vi "Scripting_AlignToConenctorPane.vi"(8 "error in":errorcluster, 11 "ViRef In":refnum<vi>) -> (0 "error out":errorcluster, 3 "VIRefOut":refnum<vi>)   [LabVIEW 2020, in "Scripting.lvclass"]
uses:
  <resource>/Framework/Providers/Open_GDS/ClassProviders/Common/ScriptingFunctions/Scripting.lvclass
  <resource>/Framework/Providers/Open_GDS/ClassProviders/Common/ScriptingFunctions/Scripting.lvclass/Scripting.ctl
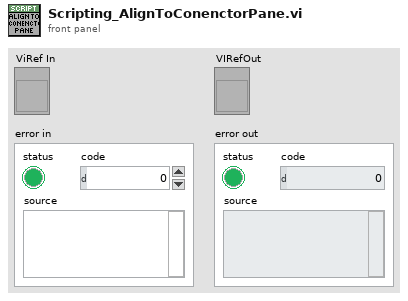
[diagram p1: front panel]
types:
  T1 = enum32{"Top Edges", "Vertical Centers", "Bottom Edges", "Left Edges", "Horizontal Centers", "Right Edges"}
  T2 = typedef "LVRectTypeDef.ctl" = cluster{"Left":i16, "Top":i16, "Right":i16, "Bottom":i16}
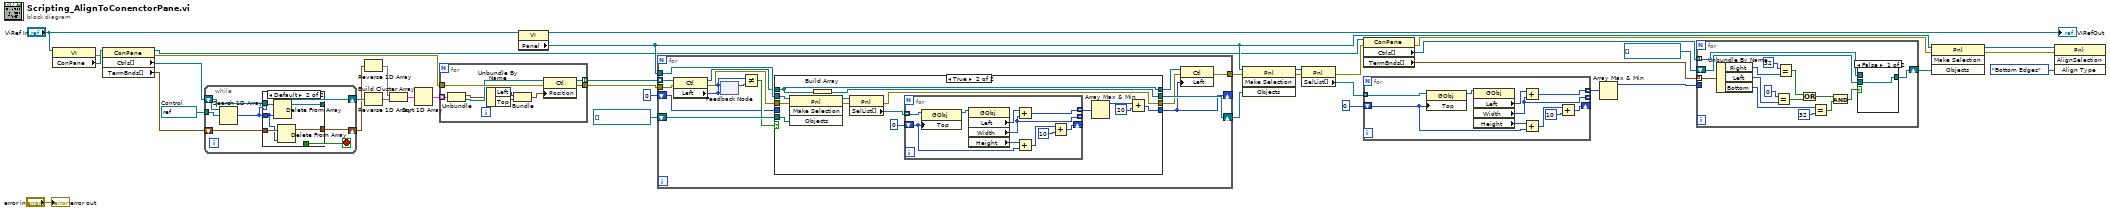
[diagram p0: block diagram]
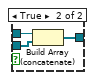
[diagram p2: hidden frame]
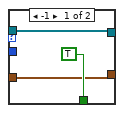
[diagram p3: hidden frame]
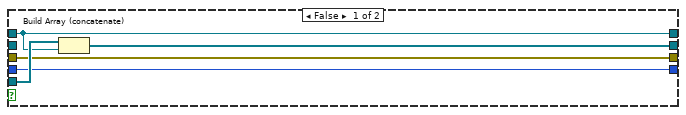
[diagram p4: hidden frame]
diagram:
  w17 = refnum<vi> refnum  # Control
  n1 = property class="VI"(reference="ViRef In") -> (error out=w28:errorcluster, "ConPane"=w33:refnum<vi>)  [unwired: 1 in, 1 out]
  n2 = property class="ConPane"(reference=w33, error in=w28) -> (reference out=w29:refnum<vi>, error out=w24:errorcluster, "Ctrls[]"=w36:refnum<vi>[], "TermBnds[]"=w35:T2[])
  n3 = while {
    tunnel: w17 -> [w39]
    shift-right: [w44] -> w27
    shift-left: w36 -> [w45]
    shift-right: [w40] -> w26
    shift-left: w35 -> [w41]
    stop <- w42 stop-if-true
    n4 = Search 1D Array(1D array=w45, element=w39) -> (index of element=w43:i32)  [unwired: 1 in]
    n5 = case shown="Default" w43 {
      tunnel: w43 -> [_ w49]
      tunnel: w45 -> [w48 w53]
      tunnel: [w48 w52] -> w44
      tunnel: [TRUE _] -> w42
      tunnel: w41 -> [w46 w51]
      tunnel: [w46 w50] -> w40
      frame -1 {
      }
      frame Default {
        n6 = Delete From Array(array=w53, index=w49) -> (array with subset deleted=w52:refnum<vi>[])  [unwired: 1 in, 1 out]
        n7 = Delete From Array(array=w51, index=w49) -> (array with subset deleted=w50:T2[])  [unwired: 1 in, 1 out]
      }
    }
  }
  n8 = Reverse 1D Array(array=w26) -> (reversed array=w21:T2[])
  n9 = Reverse 1D Array(array=w27) -> (reversed array=w20:refnum<vi>[])
  n10 = Build Cluster Array(w21, w20) -> (w19:cluster{"Rectangle":T2, refnum<vi>}[])
  n11 = Sort 1D Array(array=w19) -> (sorted array=w18:cluster{"Rectangle":T2, refnum<vi>}[])
  n12 = for {
    tunnel: [w59] -> w37 mode=indexing
    tunnel: [w58] -> w30
    tunnel: w24 -> [w57]
    tunnel: w18 -> [w56] mode=indexing
    n13 = Unbundle(w56) -> ("Rectangle"=w54:T2, w55:refnum<vi>)
    n14 = Unbundle By Name(w54) -> ("Left"=w62:i16, "Top"=w61:i16)
    n15 = Bundle("Left"=w62, "Top"=w61) -> (w60:cluster{"Left":i16, "Top":i16})  [unwired: 1 in]
    n16 = property class="Ctl"(reference=w55, error in=w57, "Position"=w60) -> (reference out=w59:refnum<vi>, error out=w58:errorcluster)
  }
  n17 = property class="VI"(reference="ViRef In") -> (reference out=→"VIRefOut":refnum<vi>, "Panel"=w32:refnum<vi>)  [unwired: 1 in, 1 out]
  n18 = for {
    shift-right: [w76] -> w22
    shift-left: refnum<vi>[] [] -> [w75]
    shift-right: [w69] -> _
    shift-left: u32 0 ("Numeric") -> [w70]
    tunnel: w32 -> [w74]
    tunnel: w37 -> [w73] mode=indexing
    tunnel: [w67] -> w31
    tunnel: w30 -> [w65]
    n19 = property class="Ctl"(reference=w73, error in=w65) -> (reference out=w64:refnum<vi>, error out=w66:errorcluster, "Left"=w71:i32)
    n20 = feedback-in #1(w71) -> ()
    n21 = feedback #1(w71) -> (w77:i32)
    n22 = Not Equal?(x=w71, y=w77) -> (x != y?=w72:bool)
    n23 = case shown="True" w72 {
      tunnel: [w82 w96] -> w76
      tunnel: w75 -> [w81 w94]
      tunnel: [w80 w89] -> w69
      tunnel: w74 -> [_ w95]
      tunnel: w70 -> [w80 _]
      tunnel: [w79 w93] -> w68
      tunnel: w66 -> [w79 w92]
      tunnel: w64 -> [w78 w91]
      tunnel: [w78 w91] -> w63
      frame False {
        n24 = Build Array (concatenate)(w81, w78) -> (w82:refnum<vi>[])
      }
      frame True {
        n25 = invoke class="Pnl" method="Make Selection"(reference=w95, error in=w92, "Objects"=w94) -> (reference out=w87:refnum<vi>, error out=w86:errorcluster)  [unwired: 1 in, 2 out]
        n26 = Build Array(w91) -> (w96:refnum<vi>[])
        n27 = property class="Pnl"(reference=w87, error in=w86) -> (error out=w93:errorcluster, "SelList[]"=w84:refnum<vi>[])  [unwired: 1 out]
        n28 = for {
          tunnel: w84 -> [w99] mode=indexing
          tunnel: [w106] -> w83 mode=indexing
          tunnel: [w105] -> _ mode=indexing
          shift-right: [w100] -> _
          shift-left: u32 0 -> [w97]
          n29 = property class="GObj"(reference=w99, "Top"=w97) -> (reference out=w98:refnum<vi>)  [unwired: 1 in, 1 out]
          n30 = property class="GObj"(reference=w98) -> ("Left"=w104:i32, "Width"=w105:u32, "Height"=w103:u32)  [unwired: 1 in, 2 out]
          n31 = Add(x=w104, y=w105) -> (x+y=w106:u32)
          n32 = Add(x=w103, y=w97) -> (x+y=w102:u32)
          n33 = Add(x=w102, y=u32 10) -> (x+y=w100:u32)
        }
        n34 = Array Max & Min(array=w83) -> (max value=w90:u32)  [unwired: 3 out]
        n35 = Add(x=w90, y=u32 20) -> (x+y=w89:u32)
      }
    }
    n36 = property class="Ctl"(reference=w63, error in=w68, "Left"=w69) -> (error out=w67:errorcluster)  [unwired: 1 out]
  }
  n37 = invoke class="Pnl" method="Make Selection"(reference=w32, error in=w31, "Objects"=w22) -> (reference out=w16:refnum<vi>, error out=w15:errorcluster)  [unwired: 1 in, 2 out]
  n38 = property class="Pnl"(reference=w16, error in=w15) -> (error out=w3:errorcluster, "SelList[]"=w13:refnum<vi>[])  [unwired: 1 out]
  n39 = property class="ConPane"(reference=w29, error in=w3) -> (error out=w4:errorcluster, "Ctrls[]"=w11:refnum<vi>[], "TermBnds[]"=w10:T2[])  [unwired: 1 out]
  n40 = for {
    tunnel: w13 -> [w109] mode=indexing
    tunnel: [w116] -> w12 mode=indexing
    tunnel: [w115] -> _ mode=indexing
    shift-right: [w110] -> _
    shift-left: u32 0 -> [w107]
    n41 = property class="GObj"(reference=w109, "Top"=w107) -> (reference out=w108:refnum<vi>)  [unwired: 1 in, 1 out]
    n42 = property class="GObj"(reference=w108) -> ("Left"=w114:i32, "Width"=w115:u32, "Height"=w113:u32)  [unwired: 1 in, 2 out]
    n43 = Add(x=w114, y=w115) -> (x+y=w116:u32)
    n44 = Add(x=w113, y=w107) -> (x+y=w112:u32)
    n45 = Add(x=w112, y=u32 10) -> (x+y=w110:u32)
  }
  n46 = Array Max & Min(array=w12) -> (max value=w2:u32)  [unwired: 3 out]
  n47 = for {
    tunnel: w11 -> [w120] mode=indexing
    tunnel: w10 -> [w131] mode=indexing
    shift-right: [w119] -> w8
    shift-left: refnum<vi>[] [] -> [w118]
    tunnel: w2 -> [_]
    n48 = Unbundle By Name(w131) -> ("Right"=w126:i16, "Left"=w128:i16, "Bottom"=w130:i16)
    n49 = Equal?(x=i16 0, y=w128) -> (x = y?=w123:bool)
    n50 = Equal?(x=i16 32 ("right"), y=w126) -> (x = y?=w124:bool)
    n51 = Or(x=w124, y=w123) -> (x .or. y?=w122:bool)
    n52 = Equal?(x=w130, y=i16 32) -> (x = y?=w121:bool)
    n53 = And(x=w122, y=w121) -> (x .and. y?=w117:bool)
    n54 = case shown="False" w117 {
      tunnel: w120 -> [_ w135]
      tunnel: [w132 w134] -> w119
      tunnel: w118 -> [w132 w133]
      frame False {
      }
      frame True {
        n55 = Build Array (concatenate)(w135, w133) -> (w134:refnum<vi>[])
      }
    }
  }
  n56 = invoke class="Pnl" method="Make Selection"(reference=w32, error in=w4, "Objects"=w8) -> (reference out=w7:refnum<vi>, error out=w5:errorcluster)  [unwired: 1 in, 2 out]
  n57 = invoke class="Pnl" method="AlignSelection"(reference=w7, error in=w5, "Align Type"=T1."Bottom Edges") -> ()  [unwired: 1 in, 4 out]
  "error out" <- "error in"
